vi "Page Source.vi"() -> ()   [LabVIEW 2020]
uses:
  C:/Users/Simon/Documents/GitHub/LV-WebView2/Source/Libs/Microsoft.Web.WebView2.WinForms.dll
  Libs/Microsoft.Web.WebView2.WinForms.dll
  Webview2 Lib/WebView2 Control Object/Register Events.vi
  Webview2 Lib/WebView2 Control Object/Read Document Source.vi
  Webview2 Lib/WebView2 Control Object/WebView2 Control.lvclass
panel:
  in  "WebView2":refnum<k24>(container)
  out "Document Source":string
  in  "stop":bool
  in  "Navigate":bool
  in  "URL":string="http://ni.com"
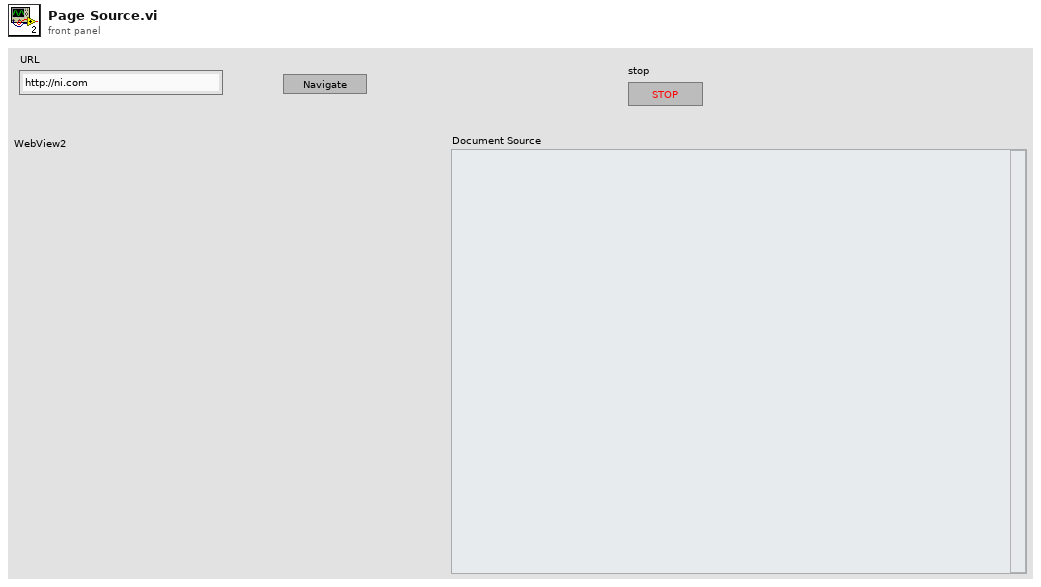
[diagram p1: front panel]
types:
  T1 = typedef "WebView2.lvlib/WebView2 Control.lvclass/Events.ctl" = cluster{"Navigation Complete Event":refnum<user-event>, "Source Changed Event":refnum<user-event>, "Document Title Changed Event":refnum<user-event>, "Status Bar Text Changed":refnum<user-event>, "Web Message Received":refnum<user-event>, "Window Close Requested":refnum<user-event>, "DOM Loaded":refnum<user-event>, "Navigation Started Event":refnum<user-event>}
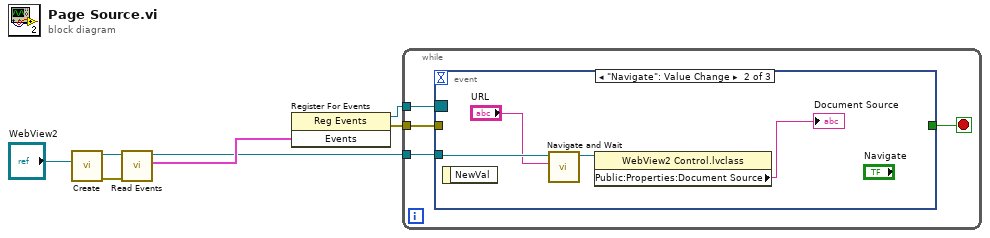
[diagram p0: block diagram]
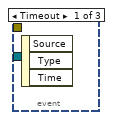
[diagram p2: hidden frame]
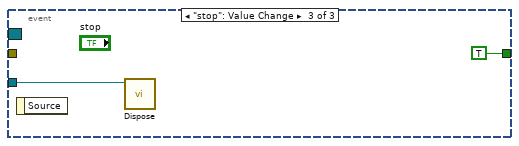
[diagram p3: hidden frame]
diagram:
  n1 = call "Create.vi"("WebView2 Control"="WebView2") -> ("error out"=w3:errorcluster, "WebView2 Control out"=w4:refnum<class "WebView2 Control.lvclass">)  [unwired: 9 in]
  n2 = call "Read Events.vi"("error in (no error)"=w3, "WebView2 Control in"=w4) -> ("Events"=w2:T1, "WebView2 Control out"=w1:refnum<class "WebView2 Control.lvclass">)  [unwired: 7 in, 1 out]
  n3 = register-events(w2) -> (reference out=w7:refnum<event-registration>, error out=w6:errorcluster)  [unwired: 2 in]
  n4 = while {
    tunnel: w7 -> [w11]
    tunnel: w6 -> [w10]
    tunnel: w1 -> [w8]
    stop <- w9 stop-if-true
    n5 = event shown="[1] \"Navigate\": Value Change" {
      selector: w11 -> [_ _ _]
      dyn-events: _ -> [_ _ _]
      timeout: _ -> [_ _ _]
      tunnel: w10 -> [_ _ _]
      tunnel: [_ _ TRUE] -> w9
      tunnel: w8 -> [_ w15 w16]
      event Timeout {
        n6 = event-data() -> ()  [unwired: 1 in, 3 out]
      }
      event "Navigate": Value Change {
        n7 = event-data() -> ()  [unwired: 1 in, 1 out]
        n8 = call "Navigate and Wait.vi"("Source"="URL", "WebView2 Control in"=w15) -> ("WebView2 Control out"=w13:refnum<class "WebView2 Control.lvclass">)  [unwired: 7 in, 2 out]
        n9 = property class="WebView2 Control.lvclass"(reference=w13) -> ("Public:Properties:Document Source"=→"Document Source":string)  [unwired: 1 in, 2 out]
      }
      event "stop": Value Change {
        n10 = event-data() -> ()  [unwired: 1 in, 1 out]
        n11 = call "Dispose.vi"("WebView2 Control in"=w16) -> ()  [unwired: 10 in, 1 out]
      }
    }
  }
